vi "Timing-calle.vi"(7 "Name (\"\" to Use UUID)":string="Event CSM Tiny") -> ()   [LabVIEW 2018]
doc: "Compact code template used to create a CSM module with a user interface. This template includes a user Event Structure for responding to user actions. The functionality of this template is identical to the CSM User Interface(UI) Module Template VI.\n\n\n> [!NOTE] <b>CSM Naming Rules</b>\n>\n> - CSM module name must be unique. Otherwise, CSM enters a `Critical Error` state.\n> - If the input module name is an empty string (\"\"), the system uses a UUID as the module name. Such a module is marked as standalone mode and does not appear in the module list.\n> - Worker Mode Rule: If the input module name ends with `#`, a worker mode node will be instantiated. Multiple worker mode nodes can form a worker mode module.\n> - Chain of Responsibility Mode Rule: If the input module name ends with `$` followed by a number, a chain of responsibility mode node will be instantiated. Multiple chain of responsibility mode nodes can form a chain of responsibility mode module.\n> - System-Level Module Rule: If the input module name starts with `.`, the module is a system-level module. Under default settings, such modules are not listed by the CSM - List Modules VI and are suitable for instantiating modules that run in the background.\n> - Submodule Rule: `.` is also allowed in a module name to separate the module name into multiple parts. CSM does not have strict rules for submodules. The `.` in the module name only marks the logical relationship between different modules. From an execution perspective, they are considered independent modules. The only difference is that you can obtain a list of logical submodules via the CSM - List Submodules VI.\n\n\n-- <b>Controls</b> --\n- <b>Name (\"\" to use UUID)</b>: CSM module name. Refer to <b>CSM Naming Rules</b> for module naming rules."
uses:
  <userlib>/_NEVSTOP/Communicable State Machine(CSM)/_Support/Typedef/_CSM_MODE.ctl
  b2fcfacf-e23a-485d-90fb-d9cb35f9c31f.vi
  <userlib>/_NEVSTOP/Communicable State Machine(CSM)/AdvanceAPI/CSM - Revert Arguments-Safe String.vi
  <userlib>/_NEVSTOP/Communicable State Machine(CSM)/_Shared/Trim Single-line Text.vi
  <userlib>/_NEVSTOP/Communicable State Machine(CSM)/AdvanceAPI/CSM - Make String Arguments Safe.vi
  <userlib>/_NEVSTOP/Communicable State Machine(CSM)/AdvanceAPI/CSM - Break Down Multiple States String.vi
  <userlib>/_NEVSTOP/Communicable State Machine(CSM)/AdvanceAPI/CSM - Compact Multiple States.vi
  <userlib>/_NEVSTOP/Communicable State Machine(CSM)/AdvanceAPI/CSM - Keywords.vi
  <userlib>/_NEVSTOP/Communicable State Machine(CSM)/addons/API-String-Arugments-Support/_Support/Data To API String Arguments.vi
  <userlib>/_NEVSTOP/Communicable State Machine(CSM)/_Polymophic/Build Asynchronous Message with Arguments.vi
  <userlib>/_NEVSTOP/Communicable State Machine(CSM)/Communicable State Machine.lvlib
panel:
  out "输出簇":T2(array[cluster])
  in  "Time":i32
  in  "Send":bool
  out "Return measage":string
  out "State History":string
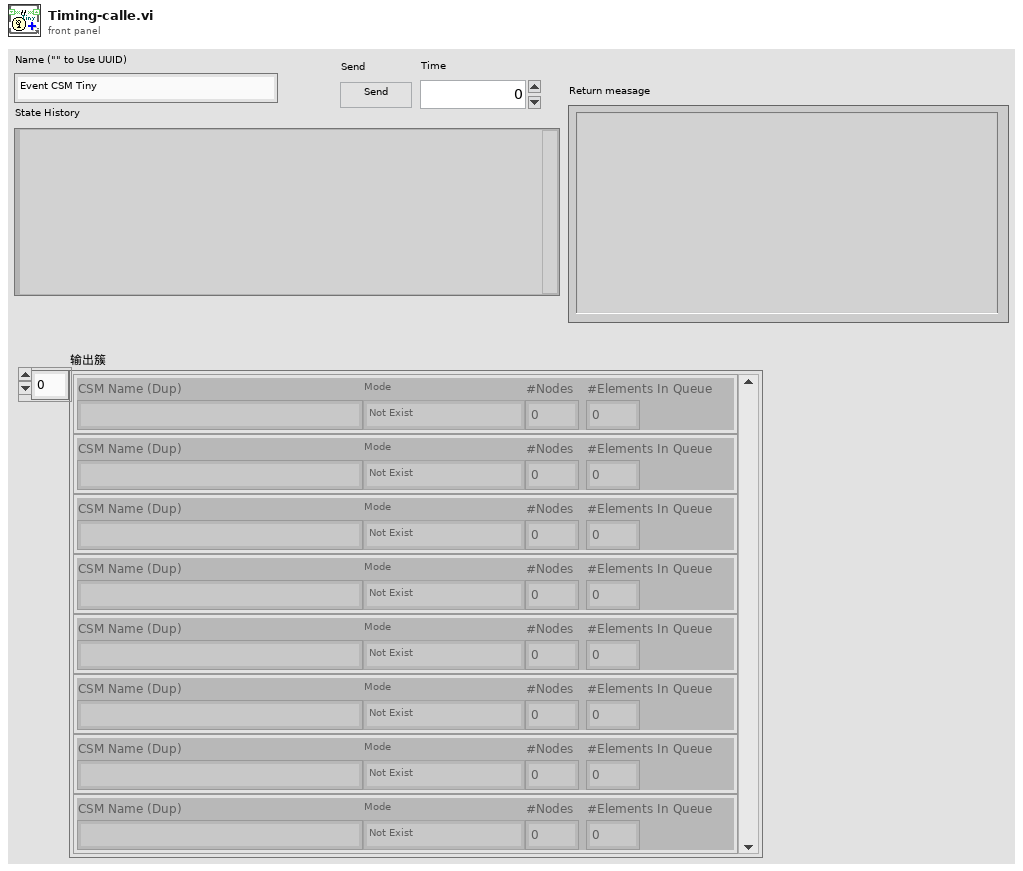
[diagram p1: front panel]
types:
  T1 = typedef "Communicable State Machine.lvlib/_CSM_MODE.ctl" = enum16{"Not Exist", "Stand Alone", "CSM", "Worker", "Worker Agent", "Chain Node", "Chain"}
  T2 = cluster{"CSM Name (Dup)":string, "Mode":T1, "#Nodes":i32, "#Elements In Queue":i32}[]
  T3 = enum32{"Invalid", "Standard", "Closed", "Hidden", "Minimized", "Maximized"}
  T4 = enum32{"invalid app kind", "Development System", "Run Time System", "Student Edition", "Embedded LabVIEW", "Evaluation", "Custom"}
  T5 = typedef "Communicable State Machine.lvlib/_CSM_Response Source Message.ctl" = cluster{"‘State":string, "’Arguments":string, "’Error":errorcluster}
  T6 = cluster{"Current VI Reference":refnum<vi>, "Close Panel on Exit?":bool}
  T7 = cluster{"Core":cluster{"Current VI Reference":refnum<vi>, "Close Panel on Exit?":bool}, "Your Boolean data":bool, "Your string data":string}
  T8 = cluster{"CSM Name (Dup)":string, "Mode":T1, "#Nodes":i32, "#Elements In Queue":i32}
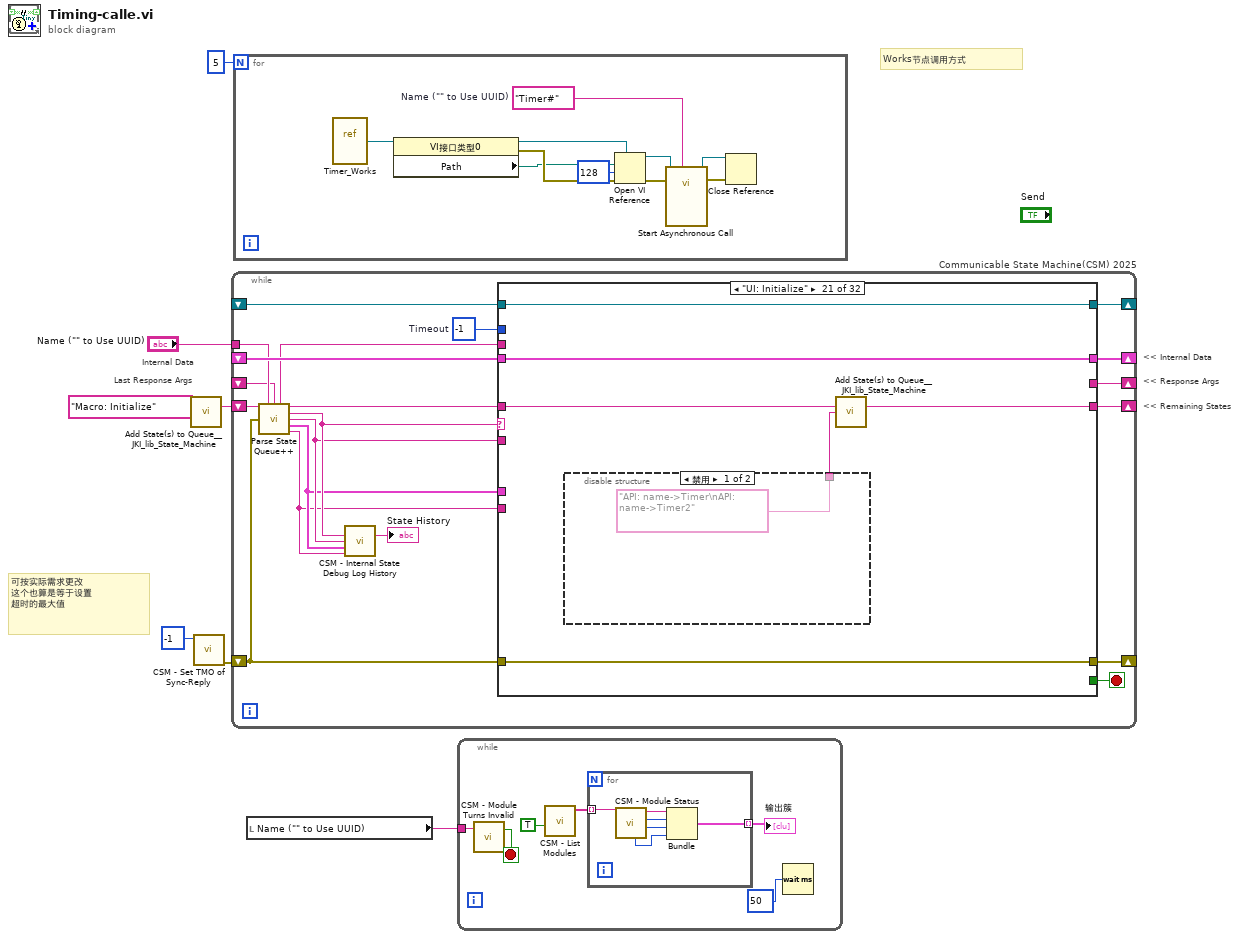
[diagram p0: block diagram]
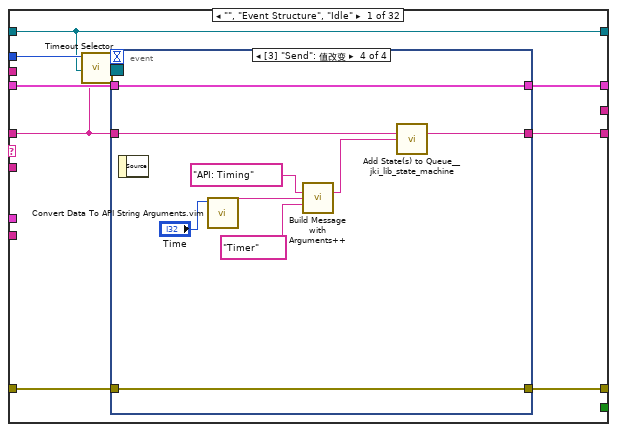
[diagram p2: hidden frame]
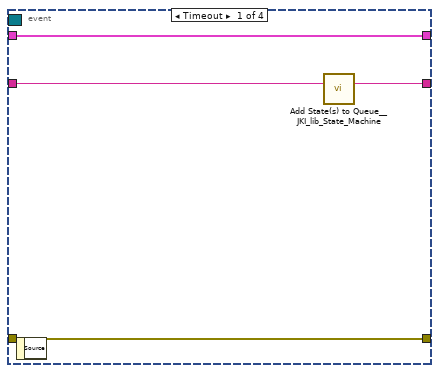
[diagram p3: hidden frame]
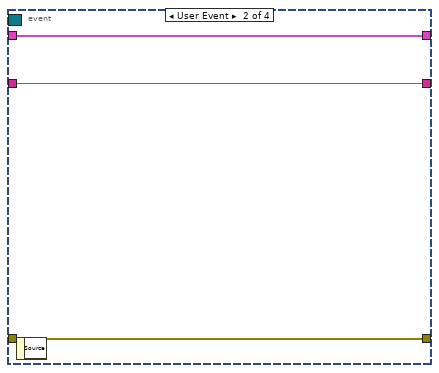
[diagram p4: hidden frame]
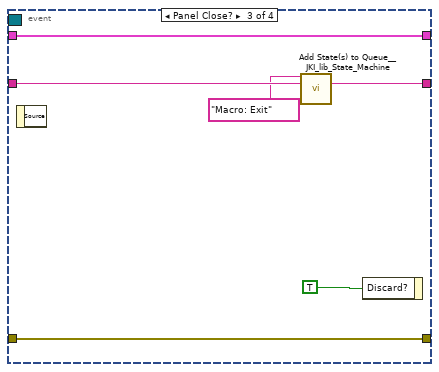
[diagram p5: hidden frame]
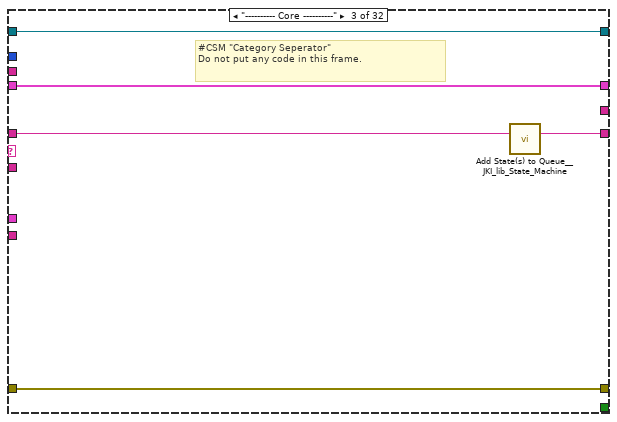
[diagram p7: hidden frame]
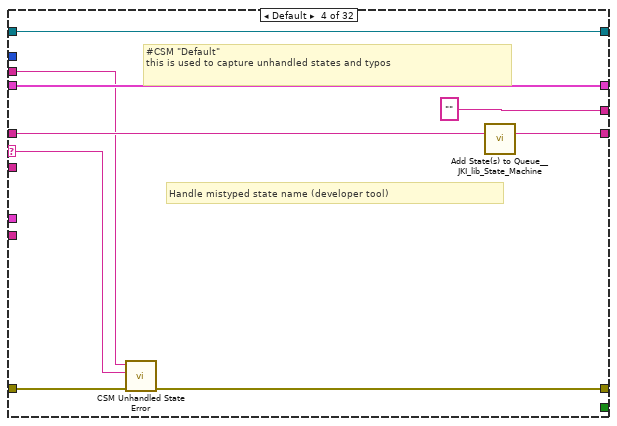
[diagram p8: hidden frame]
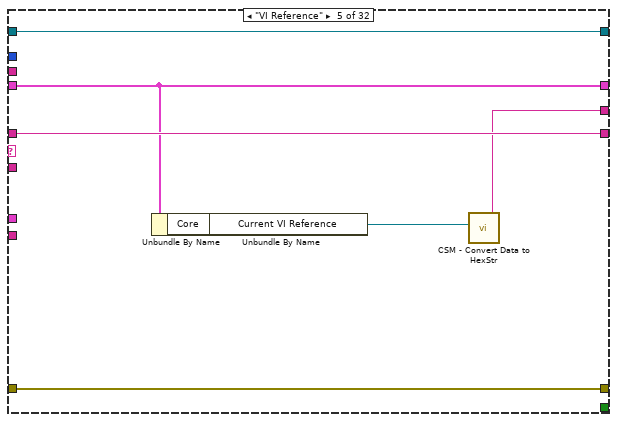
[diagram p9: hidden frame]
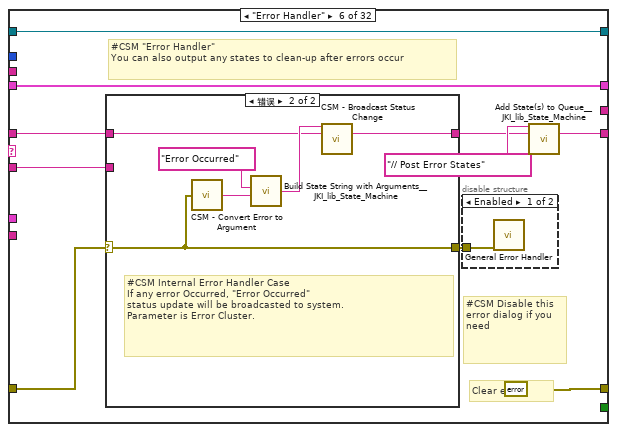
[diagram p10: hidden frame]
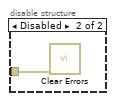
[diagram p11: hidden frame]
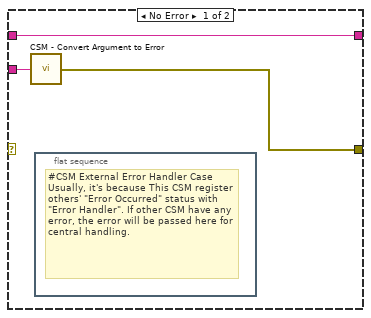
[diagram p12: hidden frame]
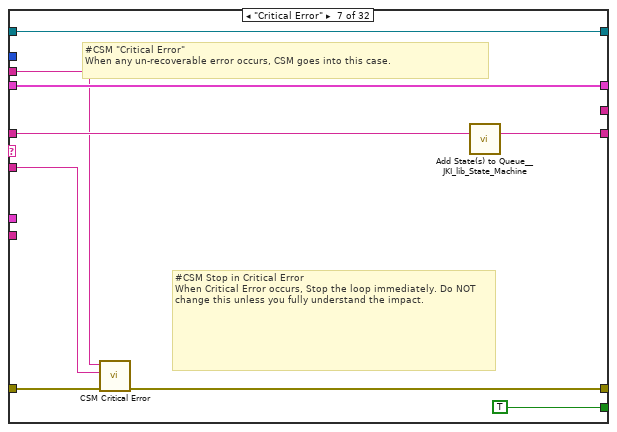
[diagram p13: hidden frame]
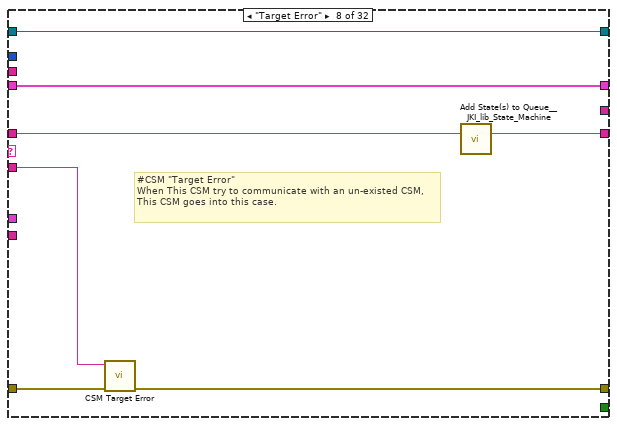
[diagram p14: hidden frame]
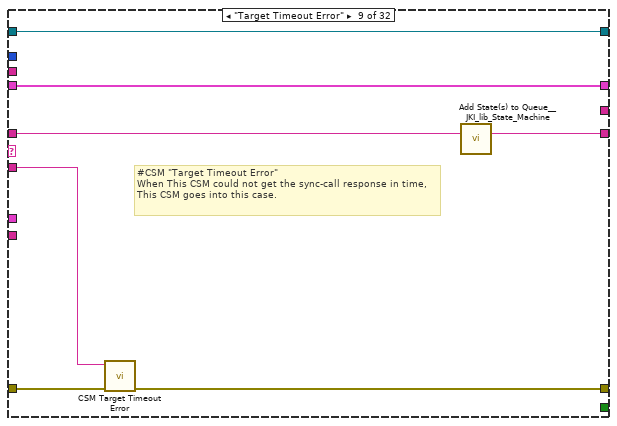
[diagram p15: hidden frame]
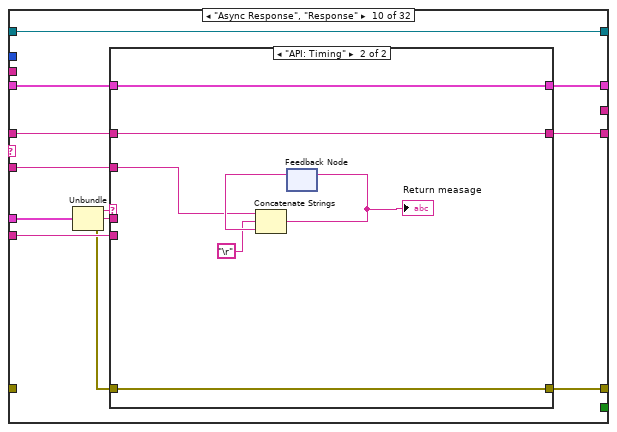
[diagram p16: hidden frame]
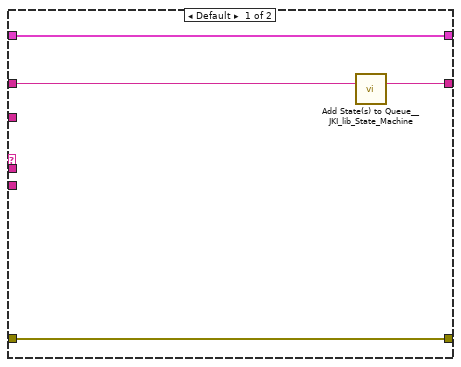
[diagram p17: hidden frame]
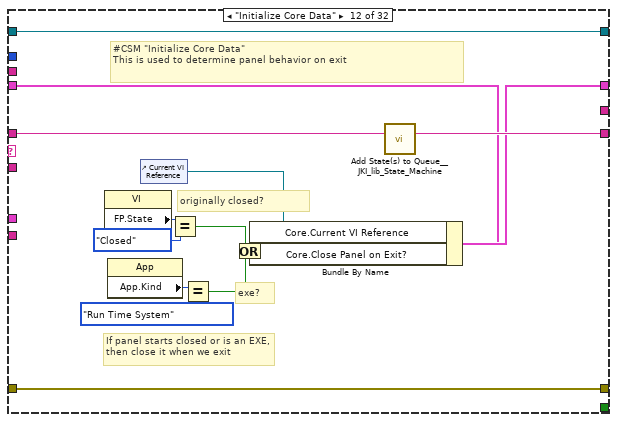
[diagram p19: hidden frame]
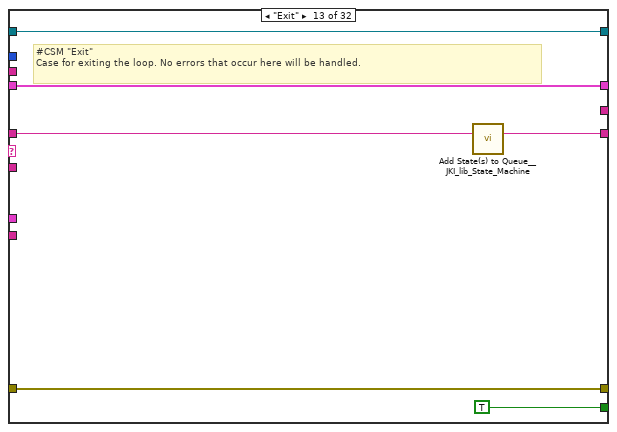
[diagram p20: hidden frame]
diagram:
  # "可按实际需求更改\n这个也算是等于设置\n超时的最大值"
  # "Works节点调用方式"
  # "Last Response Args"
  # "Internal Data"
  # "<< Internal Data"
  # "<< Response Args"
  # "<< Remaining States"
  n1 = call <vilib>:"Add State(s) to Queue__JKI_lib_State_Machine.vi"("State(s) in (\"\")"="Macro: Initialize" ("Init State(\"Macro: Initialize\")")) -> ("States Out"=w7:string)  [unwired: 14 in]
  n2 = call <userlib>:"CSM - Set TMO of Sync-Reply.vi"("TMO For Sync-Rep (ms) In"=-1) -> ("error out"=w3:errorcluster)  [unwired: 9 in, 1 out]
  n3 = while "Communicable State Machine(CSM) 2025" {
    shift-right: [w22] -> _
    shift-left: _ -> [w21]
    shift-right: [w25] -> _
    shift-left: w3 -> [w19]
    shift-right: [w24] -> _
    shift-left: w7 -> [w26]
    tunnel: "Name (\"\" to Use UUID)" -> [w15]
    shift-right: [w18] -> _
    shift-left: _ -> [w9]
    shift-right: [w17] -> _
    shift-left: _ -> [w16]
    stop <- w23 stop-if-true
    w20 = -1  # Timeout
    n4 = call <userlib>:"Parse State Queue++.vi"("State Queue"=w26, "Name (\"\" to Use UUID)"=w15, "Response Arguments"=w9, "Previous Error"=w19) -> ("Name Used"=w10:string, "Remaining States"=w27:string, "Current State"=w14:string, "Arguments"=w13:string, "Additional Information"=w12:T5, "Source CSM"=w11:string)  [unwired: 6 in]
    n5 = call <userlib>:"CSM - Internal State Debug Log History.vi"("State"=w14, "Arguments (\"\")"=w13, ">> Response Source Message >>"=w12, "Source (\"\")"=w11) -> ("Debug Log"=→"State History":string)  [unwired: 11 in]
    n6 = case shown="\"UI: Initialize\"" w14 {
      selector: w14 -> [_ _ _ w70 _ _ _ _ _ _ _ _ _ _ _ _ _ _ _ _ _ _ _ _ _ _ _ _ _ _ _ _]
      tunnel: w27 -> [w28 w61 w67 w75 w82 w88 w111 w117 w124 w133 w153 w168 w174 w179 w187 w194 w199 w206 w210 w216 w222 w230 w246 w316 w322 w335 w338 w343 w349 w357 w362 w367]
      tunnel: w13 -> [_ _ _ _ _ w87 w106 w116 w123 w132 _ _ _ _ _ _ _ _ _ _ _ w225 w240 _ _ _ _ _ w346 _ _ _]
      tunnel: w21 -> [w35 w60 w64 w73 w81 w92 w112 w119 w126 w135 w152 w161 w172 w176 _ w189 w196 w205 w209 w213 w220 w228 w242 w313 w319 w332 w337 w342 w348 w354 w359 w364]
      tunnel: [w34 w62 w65 w68 w83 errorcluster {"status"=FALSE, "code"=0, "source"=""} ("error out") w107 w114 w121 w138 w154 w165 w171 w177 w184 w190 w197 w200 w208 w214 w219 w226 w243 w314 w320 w333 w339 w344 w350 w355 w360 w365] -> w25
      tunnel: w19 -> [w33 w62 w65 w76 w83 w89 w113 w115 w122 _ w154 w165 w171 w177 w184 w191 w197 _ w211 w214 w219 w227 w244 w314 w320 w333 w339 w344 w350 w355 w360 w365]
      tunnel: [w36 w61 w66 w74 w82 w84 w110 w120 w127 w134 w153 w167 w173 w178 w186 w193 w198 w206 w210 w215 w221 w229 w245 w315 w321 w334 w338 w343 w349 w356 w361 w366] -> w24
      tunnel: [_ _ _ _ _ _ TRUE _ _ _ _ _ TRUE _ _ _ _ _ _ _ _ _ _ _ _ _ _ _ _ _ _ _] -> w23
      tunnel: [w32 w60 w64 w73 w81 w92 w112 w119 w126 w136 w152 w166 w172 w176 w185 w189 w196 w205 w209 w213 w220 w228 w242 w313 w319 w332 w337 w342 w348 w354 w359 w364] -> w22
      tunnel: w20 -> [w31 _ _ _ _ _ _ _ _ _ _ _ _ _ _ _ _ _ _ _ _ _ _ _ _ _ _ _ _ _ _ _]
      tunnel: w11 -> [_ _ _ _ _ _ _ _ _ w130 _ _ _ _ _ _ _ _ _ _ _ _ _ _ _ _ _ _ _ _ _ _]
      tunnel: w12 -> [_ _ _ _ _ _ _ _ _ w137 _ _ _ _ _ _ _ _ _ _ _ _ _ _ _ _ _ _ _ _ _ _]
      tunnel: [_ _ _ "" w77 _ _ _ _ _ _ _ _ _ _ _ _ _ _ _ _ _ _ _ _ _ _ "API1 Response" w345 _ _ _] -> w18
      tunnel: [w30 w59 w63 w71 w80 w91 w108 w118 w125 w139 w151 w155 w169 w175 w180 w188 w195 w204 w207 w212 w218 w224 w239 w312 w317 w325 w336 w341 w347 w353 w358 w363] -> w17
      tunnel: w16 -> [w30 w59 w63 w71 w80 w91 w108 w118 w125 w139 w151 w155 w169 w175 w180 w188 w195 _ w207 w212 w218 w224 w239 w312 w317 w325 w336 w341 w347 w353 w358 w363]
      tunnel: w10 -> [_ _ _ w69 _ _ w105 _ _ _ _ _ _ _ _ _ _ w203 _ _ _ _ _ _ _ _ _ _ _ _ _ _]
      frame "", "Event Structure", "Idle" {
        n7 = call <userlib>:"Timeout Selector.vi"("Remaining States"=w28, "Timeout Expected"=w31) -> ("Timeout"=w29:i32)  [unwired: 5 in]
        n8 = event shown="[3] \"Send\": 值改变" {
          selector: w30 -> [_ _ _ _]
          dyn-events: _ -> [_ _ _ _]
          timeout: w29 -> [_ _ _ _]
          tunnel: w28 -> [w40 w42 w49 w55]
          tunnel: [w39 w42 w48 w56] -> w36
          tunnel: w35 -> [w37 w43 w46 w57]
          tunnel: [w38 w41 w47 w58] -> w34
          tunnel: w33 -> [w38 w41 w47 w58]
          tunnel: [w37 w43 w46 w57] -> w32
          event Timeout {
            n9 = event-data() -> ()  [unwired: 1 in, 1 out]
            n10 = call <vilib>:"Add State(s) to Queue__JKI_lib_State_Machine.vi"("State(s) in (\"\")"=w40) -> ("States Out"=w39:string)  [unwired: 14 in]
          }
          event User Event {
            n11 = event-data() -> ()  [unwired: 1 in, 1 out]
          }
          event Panel Close? {
            n12 = event-data() -> ()  [unwired: 1 in, 1 out]
            n13 = call <vilib>:"Add State(s) to Queue__JKI_lib_State_Machine.vi"("State(s) in Front (\"\")"="Macro: Exit", "State(s) in (\"\")"=w49) -> ("States Out"=w48:string)  [unwired: 13 in]
            n14 = event-data("Discard?"=TRUE) -> ()  [unwired: 1 in, 1 out]
          }
          event "Send": Value Change {
            n15 = event-data() -> ()  [unwired: 1 in, 1 out]
            n16 = call "Convert Data To API String Arguments.vim"("Data"="Time") -> ("API String"=w51:string)  [unwired: 7 in, 1 out]
            n17 = call-poly <userlib>:"Build Message with Arguments++.vi"("State With Arguments"="API: Timing", "Arguments (\"\")"=w51, "Target Module (\"\")"="Timer" ("Target Module (\"\")")) -> ("CSM Message String"=w54:string)  [unwired: 12 in]
            n18 = call <vilib>:"Add State(s) to Queue__jki_lib_state_machine.vi"("State(s) in (\"\")"=w55, "State(s) at Back (\"\")"=w54) -> ("States Out"=w56:string)  [unwired: 13 in]
          }
        }
      }
      frame "CSM Documentation" {
      }
      frame "---------- Core ----------" {
        # "#CSM \"Category Seperator\"\nDo not put any code in this frame."
        n19 = call <vilib>:"Add State(s) to Queue__JKI_lib_State_Machine.vi"("State(s) in (\"\")"=w67) -> ("States Out"=w66:string)  [unwired: 14 in]
      }
      frame Default {
        # "#CSM \"Default\"\nthis is used to capture unhandled states and typos"
        # "Handle mistyped state name (developer tool)"
        n20 = call <userlib>:"CSM Unhandled State Error.vi"("error in (no error)"=w76, "Undefined State"=w70, "CSM Name"=w69) -> ("error out"=w68:errorcluster)  [unwired: 8 in]
        n21 = call <vilib>:"Add State(s) to Queue__JKI_lib_State_Machine.vi"("State(s) in (\"\")"=w75) -> ("States Out"=w74:string)  [unwired: 14 in]
      }
      frame "VI Reference" {
        n22 = Unbundle By Name(w81) -> ("Core"=w79:T6)
        n23 = Unbundle By Name(w79) -> ("Current VI Reference"=w78:refnum<vi>)
        n24 = call <userlib>:"CSM - Convert Data to HexStr.vi"("Variant"=w78) -> ("HEX String (0-9,A-F)"=w77:string)  [unwired: 8 in]
      }
      frame "Error Handler" {
        # "#CSM Disable this error dialog if you need"
        # "#CSM \"Error Handler\"\nYou can also output any states to clean-up after errors occur"
        # "Clear error"
        n25 = case shown="错误" w89 {
          selector: w89 -> [_ w99]
          tunnel: [w98 w101] -> w85
          tunnel: w88 -> [w98 w100]
          tunnel: w87 -> [w97 _]
          tunnel: [w96 w99] -> w90
          frame No Error {
            n26 = call <userlib>:"CSM - Convert Argument to Error.vi"("Argument"=w97) -> ("Error"=w96:errorcluster)  [unwired: 4 in]
            n27 = flat-sequence {
              frame #0 {
                # "#CSM External Error Handler Case\nUsually, it's because This CSM register others' \"Error Occurred\" status with \"Error Handler\". If other CSM have any error, the error will be passed here for central handling."
              }
            }
          }
          frame Error {
            # "#CSM Internal Error Handler Case \nIf any error Occurred, \"Error Occurred\" \nstatus update will be broadcasted to system.\nParameter is Error Cluster."
            n28 = call <userlib>:"CSM - Convert Error to Argument.vi"("Error"=w99) -> ("Argument"=w103:string)  [unwired: 4 in]
            n29 = call <vilib>:"Build State String with Arguments__JKI_lib_State_Machine.vi"("Arguments (\"\")"=w103, "State"="Error Occurred" ("Status with Arguments")) -> ("State with Arguments"=w102:string)  [unwired: 4 in]
            n30 = call <userlib>:"CSM - Broadcast Status Change.vi"("Status With Arguments"=w102, "State Queue"=w100) -> ("Remaining States"=w101:string)  [unwired: 13 in]
          }
        }
        n31 = disable-structure shown="Enabled" {
          disable-tunnel: w90 -> [w94 w95]
          frame Enabled {
            n32 = call <vilib>:"General Error Handler.vi"("error in (no error)"=w94) -> ()  [unwired: 10 in, 5 out]
          }
          frame Disabled {
            n33 = call <vilib>:"Clear Errors.vi"("error in (no error)"=w95) -> ()  [unwired: 5 in, 2 out]
          }
        }
        n34 = call <vilib>:"Add State(s) to Queue__JKI_lib_State_Machine.vi"("State(s) in Front (\"\")"="// Post Error States", "State(s) in (\"\")"=w85) -> ("States Out"=w84:string)  [unwired: 13 in]
      }
      frame "Critical Error" {
        # "#CSM Stop in Critical Error\nWhen Critical Error occurs, Stop the loop immediately. Do NOT change this unless you fully understand the impact."
        # "#CSM \"Critical Error\"\nWhen any un-recoverable error occurs, CSM goes into this case."
        n35 = call <userlib>:"CSM Critical Error.vi"("error in (no error)"=w113, "Arugments (As Reason)"=w106, "CSM Name"=w105) -> ("error out"=w107:errorcluster)  [unwired: 8 in]
        n36 = call <vilib>:"Add State(s) to Queue__JKI_lib_State_Machine.vi"("State(s) in (\"\")"=w111) -> ("States Out"=w110:string)  [unwired: 14 in]
      }
      frame "Target Error" {
        # "#CSM \"Target Error\"\nWhen This CSM try to communicate with an un-existed CSM, This CSM goes into this case."
        n37 = call <userlib>:"CSM Target Error.vi"("error in (no error)"=w115, "Arguments (As CSM Name)"=w116) -> ("error out"=w114:errorcluster)  [unwired: 9 in]
        n38 = call <vilib>:"Add State(s) to Queue__JKI_lib_State_Machine.vi"("State(s) in (\"\")"=w117) -> ("States Out"=w120:string)  [unwired: 14 in]
      }
      frame "Target Timeout Error" {
        # "#CSM \"Target Timeout Error\"\nWhen This CSM could not get the sync-call response in time, This CSM goes into this case."
        n39 = call <userlib>:"CSM Target Timeout Error.vi"("error in (no error)"=w122, "Arguments (As CSM Name)"=w123) -> ("error out"=w121:errorcluster)  [unwired: 9 in]
        n40 = call <vilib>:"Add State(s) to Queue__JKI_lib_State_Machine.vi"("State(s) in (\"\")"=w124) -> ("States Out"=w127:string)  [unwired: 14 in]
      }
      frame "Async Response", "Response" {
        n41 = Unbundle(w137) -> ("‘State"=w131:string, "’Arguments"=w129:string, "’Error"=w128:errorcluster)
        n42 = case shown="\"API: Timing\"" w131 {
          tunnel: [w143 w150] -> w138
          tunnel: w128 -> [w143 w150]
          tunnel: [w142 w149] -> w136
          tunnel: w135 -> [w142 w149]
          tunnel: [w140 w148] -> w134
          tunnel: w133 -> [w141 w148]
          tunnel: w132 -> [_ w144]
          tunnel: w130 -> [_ _]
          tunnel: w129 -> [_ _]
          frame Default {
            n43 = call <vilib>:"Add State(s) to Queue__JKI_lib_State_Machine.vi"("State(s) in (\"\")"=w141) -> ("States Out"=w140:string)  [unwired: 14 in]
          }
          frame "API: Timing" {
            n44 = feedback #1() -> (w147:string)  [unwired: 1 in]
            n45 = Concatenate Strings(w144, "\r", w147) -> (w145:string)
            "Return measage" <- w145
            n46 = feedback-in #1(w145) -> ()
          }
        }
      }
      frame "Async Message Posted" {
      }
      frame "Initialize Core Data" {
        # "#CSM \"Initialize Core Data\"\nThis is used to determine panel behavior on exit"
        # "originally closed?"
        # "exe?"
        # "If panel starts closed or is an EXE, then close it when we exit"
        n47 = property class="VI"() -> ("FP.State"=w158:T3)  [unwired: 2 in, 2 out]
        n48 = property class="App"() -> ("App.Kind"=w164:T4)  [unwired: 2 in, 2 out]
        n49 = control-ref of="Current VI Reference"() -> (w159:refnum<vi>)
        n50 = Equal?(x=w158, y=T3."Closed" ("Front Panel Window:State")) -> (x = y?=w156:bool)
        n51 = Equal?(x=w164, y=T4."Run Time System" ("Application:Kind")) -> (x = y?=w162:bool)
        n52 = Or(x=w156, y=w162) -> (x .or. y?=w160:bool)
        n53 = Bundle By Name(cluster=w161, "Core.Current VI Reference"=w159, "Core.Close Panel on Exit?"=w160) -> (w166:T7)
        n54 = call <vilib>:"Add State(s) to Queue__JKI_lib_State_Machine.vi"("State(s) in (\"\")"=w168) -> ("States Out"=w167:string)  [unwired: 14 in]
      }
      frame "Exit" {
        # "#CSM \"Exit\"\nCase for exiting the loop. No errors that occur here will be handled."
        n55 = call <vilib>:"Add State(s) to Queue__JKI_lib_State_Machine.vi"("State(s) in (\"\")"=w174) -> ("States Out"=w173:string)  [unwired: 14 in]
      }
      frame "---------- Data ----------" {
        # "#CSM \"Category Seperator\"\nDo not put any code in this frame."
        n56 = call <vilib>:"Add State(s) to Queue__JKI_lib_State_Machine.vi"("State(s) in (\"\")"=w179) -> ("States Out"=w178:string)  [unwired: 14 in]
      }
      frame "Data: Initialize" {
        w181 = T6 {"Current VI Reference"=refnum, "Close Panel on Exit?"=FALSE}  # Core
        w183 = TRUE  # Your Boolean data
        w182 = ""  # Your string data
        # "#CSM do not delete - used by framework"
        # "#CSM Expand Bundle to add new data elements to shift register data."
        # "#CSM Add new data here."
        # "Initialize the shift-register data, here.\n(data names are defined by what you wire into the bundle function)"
        n57 = Bundle("Core"=w181, "Your Boolean data"=w183, "Your string data"=w182) -> (w185:T7)  [unwired: 1 in]
        n58 = call <vilib>:"Add State(s) to Queue__JKI_lib_State_Machine.vi"("State(s) in (\"\")"=w187) -> ("States Out"=w186:string)  [unwired: 14 in]
      }
      frame "Data: Cleanup" {
        # "Cleanup any data and references, here.\n(this is called automatically, by the Macro: Exit)"
        n59 = Unbundle By Name(w189) -> ("Core.Current VI Reference"=w192:refnum<vi>)
        n60 = Close Reference(reference=w192, error in (no error)=w191) -> (error out=w190:errorcluster)
        n61 = call <vilib>:"Add State(s) to Queue__JKI_lib_State_Machine.vi"("State(s) in (\"\")"=w194) -> ("States Out"=w193:string)  [unwired: 14 in]
      }
      frame "---------- Events ----------" {
        # "#CSM \"Category Seperator\"\nDo not put any code in this frame."
        n62 = call <vilib>:"Add State(s) to Queue__JKI_lib_State_Machine.vi"("State(s) in (\"\")"=w199) -> ("States Out"=w198:string)  [unwired: 14 in]
      }
      frame "Events: Register" {
        # "#CSM \"Events: Register\"\nRegister user event. New Message Event is registered to break CSM waiting in event structure by default."
        # "#CSM Register New Message Event\nRegister message event to break Waiting in Event structure."
        n63 = call <userlib>:"CSM - Get New State Notifier Event.vi"("Name (\"\" to Use UUID)"=w203) -> ("error out"=w201:errorcluster, "New State Notifier Event"=w202:refnum<user-event>)  [unwired: 9 in]
        n64 = register-events(error in=w201, w202) -> (reference out=w204:refnum<event-registration>, error out=w200:errorcluster)  [unwired: 1 in]
      }
      frame "Events: Unregister" {
        # "#CSM \"Events: Unregister\"\nUnregister user event."
        n65 = Unregister For Events(event registration refnum=w207, error in=w211) -> (error out=w208:errorcluster)
      }
      frame "---------- UI ----------" {
        # "#CSM \"Category Seperator\"\nDo not put any code in this frame."
        n66 = call <vilib>:"Add State(s) to Queue__JKI_lib_State_Machine.vi"("State(s) in (\"\")"=w216) -> ("States Out"=w215:string)  [unwired: 14 in]
      }
      frame "UI: Initialize" {
        n67 = disable-structure shown="禁用" {
          disable-tunnel: ["API: name->Timer\nAPI: name->Timer2" ("State(s) in Front (\"\")") _] -> w217
          frame Disabled {
          }
          frame Enabled {
          }
        }
        n68 = call <vilib>:"Add State(s) to Queue__JKI_lib_State_Machine.vi"("State(s) in (\"\")"=w222, "State(s) at Back (\"\")"=w217) -> ("States Out"=w221:string)  [unwired: 13 in]
      }
      frame "UI: Cursor Set" {
        # "#CSM \"UI: Cursor Set\"\nSet and Unset Cursor Busy.\n(Usage: \"UI: Cursor Set >> Busy|Idle\")"
        # "Argument"
        n69 = disable-structure shown="Default" {
          disable-tunnel: w227 -> [w233 w238]
          disable-tunnel: [w232 w238] -> w226
          disable-tunnel: w225 -> [w231 _]
          frame condition #0 (active) {
            n70 = case shown="\"Idle\", 默认" w231 {
              tunnel: w233 -> [w235 w237]
              tunnel: [w234 w236] -> w232
              frame "Idle", Default {
                n71 = call <vilib>:"Unset Busy.vi"("error in (no error)"=w235) -> ("error out"=w234:errorcluster)  [unwired: 10 in]
              }
              frame "Busy" {
                n72 = call <vilib>:"Set Busy.vi"("error in (no error)"=w237) -> ("error out"=w236:errorcluster)  [unwired: 9 in, 1 out]
              }
            }
          }
          frame condition #1 {
          }
        }
        n73 = call <vilib>:"Add State(s) to Queue__JKI_lib_State_Machine.vi"("State(s) in (\"\")"=w230) -> ("States Out"=w229:string)  [unwired: 14 in]
      }
      frame "UI: Front Panel State" {
        # "#CSM \"UI: Front Panel State\"\nSet Front Panel Open or Closed\n(Usage: \"UI: Front Panel State >> Open|Close\")"
        # "Argument"
        n74 = Unbundle By Name(w242) -> ("Core.Current VI Reference"=w241:refnum<vi>)
        n75 = call <vilib>:"Add State(s) to Queue__JKI_lib_State_Machine.vi"("State(s) in (\"\")"=w246) -> ("States Out"=w245:string)  [unwired: 14 in]
        n76 = case shown="\"Close\", \"Closed\"" w240 {
          tunnel: w244 -> [w252 w267 w278 w291 w304]
          tunnel: [w254 w268 w280 w293 w306] -> w243
          tunnel: w241 -> [w253 w265 w279 w292 w305]
          frame "Open", "Standard", Default {
            w247 = T3."Standard" ("State")
            n77 = property class="VI"(reference=w253, error in=w252) -> (reference out=w250:refnum<vi>, error out=w251:errorcluster, "FP.State"=w249:T3)
            n78 = Not Equal?(x=w249, y=w247) -> (x != y?=w248:bool)
            n79 = case shown="真" w248 {
              tunnel: [w258 w260] -> w254
              tunnel: w251 -> [w257 w260]
              tunnel: w250 -> [w256 _]
              tunnel: w247 -> [w255 _]
              frame True {
                n80 = invoke class="VI" method="FP.Open"(reference=w256, error in=w257, "Activate"=TRUE, "State"=w255) -> (error out=w258:errorcluster)  [unwired: 1 in, 4 out]
              }
              frame False {
              }
            }
          }
          frame "Close", "Closed" {
            n81 = property class="VI"(reference=w265, error in=w267) -> (reference out=w264:refnum<vi>, error out=w266:errorcluster, "FP.State"=w262:T3)
            n82 = Not Equal?(x=w262, y=T3."Closed" ("Front Panel Window:State")) -> (x != y?=w261:bool)
            n83 = case shown="假" w261 {
              tunnel: [w269 w272] -> w268
              tunnel: w266 -> [w269 w271]
              tunnel: w264 -> [_ w270]
              frame False {
              }
              frame True {
                n84 = invoke class="VI" method="FP.Close"(reference=w270, error in=w271) -> (error out=w272:errorcluster)  [unwired: 1 in, 2 out]
              }
            }
          }
          frame "Hidden", "Hide" {
            w273 = T3."Hidden" ("State")
            n85 = property class="VI"(reference=w279, error in=w278) -> (reference out=w276:refnum<vi>, error out=w277:errorcluster, "FP.State"=w275:T3)
            n86 = Not Equal?(x=w275, y=w273) -> (x != y?=w274:bool)
            n87 = case shown="真" w274 {
              tunnel: [w284 w285] -> w280
              tunnel: w277 -> [w283 w285]
              tunnel: w276 -> [w282 _]
              tunnel: w273 -> [w281 _]
              frame True {
                n88 = invoke class="VI" method="FP.Open"(reference=w282, error in=w283, "State"=w281) -> (error out=w284:errorcluster)  [unwired: 2 in, 4 out]
              }
              frame False {
              }
            }
          }
          frame "Minimize", "Minimized" {
            w286 = T3."Minimized" ("State")
            n89 = property class="VI"(reference=w292, error in=w291) -> (reference out=w289:refnum<vi>, error out=w290:errorcluster, "FP.State"=w288:T3)
            n90 = Not Equal?(x=w288, y=w286) -> (x != y?=w287:bool)
            n91 = case shown="真" w287 {
              tunnel: [w297 w298] -> w293
              tunnel: w290 -> [w296 w298]
              tunnel: w289 -> [w295 _]
              tunnel: w286 -> [w294 _]
              frame True {
                n92 = invoke class="VI" method="FP.Open"(reference=w295, error in=w296, "State"=w294) -> (error out=w297:errorcluster)  [unwired: 2 in, 4 out]
              }
              frame False {
              }
            }
          }
          frame "Maximize", "Maximized" {
            w299 = T3."Maximized" ("State")
            n93 = property class="VI"(reference=w305, error in=w304) -> (reference out=w302:refnum<vi>, error out=w303:errorcluster, "FP.State"=w301:T3)
            n94 = Not Equal?(x=w301, y=w299) -> (x != y?=w300:bool)
            n95 = case shown="真" w300 {
              tunnel: [w310 w311] -> w306
              tunnel: w303 -> [w309 w311]
              tunnel: w302 -> [w308 _]
              tunnel: w299 -> [w307 _]
              frame True {
                n96 = invoke class="VI" method="FP.Open"(reference=w308, error in=w309, "State"=w307) -> (error out=w310:errorcluster)  [unwired: 2 in, 4 out]
              }
              frame False {
              }
            }
          }
        }
      }
      frame "---------- Macro ----------" {
        # "#CSM \"Category Seperator\"\nDo not put any code in this frame."
        n97 = call <vilib>:"Add State(s) to Queue__JKI_lib_State_Machine.vi"("State(s) in (\"\")"=w316) -> ("States Out"=w315:string)  [unwired: 14 in]
      }
      frame "Macro: Initialize" {
        w318 = "Data: Initialize\nInitialize Core Data\nEvents: Register\nUI: Initialize\nUI: Front Panel State >> Open"  # Data: Initialize Initialize Core Data Events: Register UI: Initialize UI: Front Panel State >> Open
        # "#CSM \"Macro: Initialize\"\nInitialization Macro (This is called once, when the VI starts)"
        n98 = call <vilib>:"Add State(s) to Queue__JKI_lib_State_Machine.vi"("State(s) in Front (\"\")"=w318, "State(s) in (\"\")"=w322) -> ("States Out"=w321:string)  [unwired: 13 in]
      }
      frame "Macro: Exit" {
        # "#CSM \"Macro: Exit\"\nExit Macro (This is called once, when the VI exits)"
        n99 = Unbundle By Name(w332) -> ("Core.Close Panel on Exit?"=w331:bool)
        n100 = call <userlib>:"CSM - Build Exit Messages of CSMs.vi"("CSMs"=string[] ["Timer"]) -> ("States"=w324:string)  [unwired: 14 in]
        n101 = Select(t="UI: Front Panel State >> Close", s=w331, f="") -> (s? t:f=w328:string)
        n102 = call <vilib>:"Add State(s) to Queue__JKI_lib_State_Machine.vi"("State(s) in Front (\"\")"=w324, "State(s) in (\"\")"=w328, "State(s) at Back (\"\")"="Data: Cleanup\nEvents: Unregister\nExit") -> ("States Out"=w326:string)  [unwired: 12 in]
        n103 = call <vilib>:"Add State(s) to Queue__JKI_lib_State_Machine.vi"("State(s) in Front (\"\")"=w326, "State(s) in (\"\")"=w335) -> ("States Out"=w334:string)  [unwired: 13 in]
      }
      frame "---------- API ----------" {
        # "#CSM \"Category Seperator\"\nDo not put any code in this frame."
      }
      frame "API: API1" {
        # "#CSM API Example\nCopy/Rename this case for your own API"
        # "#CSM Response\nConnect this to return the response of your API"
        # "#CSM >> Source CSM >>\nIf you need to tell who triggered this state , use this string. If it's this case itself, this string is \"\"."
        # "#CSM >> Arguments >>\nDeal with the parameter if any"
      }
      frame "API: API2" {
        # "#CSM API Example\nCopy/Rename this case for your own API"
        # "unpack Hex String  to Variant\nif complex parameter is needed."
        n104 = call <userlib>:"CSM - Convert HexStr to Data.vi"("HEX String"=w346) -> ()  [unwired: 7 in, 2 out]
        n105 = disable-structure shown="Disabled" {
          disable-tunnel: [w351 "API2 Response"] -> w345
          frame Disabled {
            # "pack variant to hexstr \nif complex response is needed."
            # "complex Response"
            n106 = call <userlib>:"CSM - Convert Data to HexStr.vi"() -> ("HEX String (0-9,A-F)"=w351:string)  [unwired: 9 in]
          }
          frame Enabled {
          }
        }
      }
      frame "---------- Action ----------" {
        # "#CSM \"Category Seperator\"\nDo not put any code in this frame."
        n107 = call <vilib>:"Add State(s) to Queue__JKI_lib_State_Machine.vi"("State(s) in (\"\")"=w357) -> ("States Out"=w356:string)  [unwired: 14 in]
      }
      frame "Action: action1" {
        # "#CSM \"Internal State\"\nThis category is used for holding internal states"
        n108 = call <vilib>:"Add State(s) to Queue__JKI_lib_State_Machine.vi"("State(s) in (\"\")"=w362) -> ("States Out"=w361:string)  [unwired: 14 in]
      }
      frame "Action: action2" {
        # "#CSM \"Internal State\"\nThis category is used for holding internal states"
        n109 = call <vilib>:"Add State(s) to Queue__JKI_lib_State_Machine.vi"("State(s) in (\"\")"=w367) -> ("States Out"=w366:string)  [unwired: 14 in]
      }
    }
  }
  n110 = for {
    N: 5 -> [_]
    w368 = "Timer#"  # Name ("" to Use UUID)
    n111 = vi-ref "Timer_Works.vi"() -> (w370:refnum<vi>)
    n112 = property class="VI接口类型0"(reference=w370) -> (reference out=w374:refnum<vi>, error out=w372:errorcluster, "Path"=w371:path)  [unwired: 1 in]
    n113 = Open VI Reference(type specifier VI Refnum (for type only)=w374, vi path=w371, options=128, error in (no error)=w372) -> (vi reference=w373:refnum<vi>, error out=w369:errorcluster)  [unwired: 2 in]
    n114 = call-by-ref "Start Asynchronous Call"(reference=w373, error in=w369, "Name(\"\" to use uuid)"=w368) -> (reference out=w376:refnum<vi>, error out=w375:errorcluster)  [unwired: 11 in]
    n115 = Close Reference(reference=w376, error in (no error)=w375) -> ()  [unwired: 1 out]
  }
  n116 = local read "Name (\"\" to Use UUID)"() -> (w1:string)
  n117 = while {
    tunnel: w1 -> [w380]
    stop <- w379 stop-if-true
    n118 = call <userlib>:"CSM - Module Turns Invalid.vi"("CSM Name"=w380) -> ("Turn Invalid (Exit)?"=w379:bool)  [unwired: 2 in]
    n119 = call <userlib>:"CSM - List Modules.vi"("With Nodes? (F)"=TRUE) -> ("Module Names"=w383:string[])  [unwired: 9 in, 1 out]
    n120 = for {
      tunnel: w383 -> [w389] mode=indexing
      tunnel: [w384] -> w382 mode=indexing
      n121 = call <userlib>:"CSM - Module Status.vi"("CSM Name"=w389) -> ("#Nodes"=w386:i32, "Mode"=w387:T1, "CSM Name (Dup)"=w388:string, "#Elements In Queue"=w385:i32)  [unwired: 6 in, 1 out]
      n122 = Bundle("CSM Name (Dup)"=w388, "Mode"=w387, "#Nodes"=w386, "#Elements In Queue"=w385) -> (w384:T8)  [unwired: 1 in]
    }
    "输出簇" <- w382
    n123 = Wait (ms)(milliseconds to wait=u32 50 ("等待时间（毫秒）")) -> ()  [unwired: 1 out]
  }
